vi "Alarm_Pattern_Control.vi"(0 "error in (no error)":errorcluster caption="错误输入（无错误）", 2 "Tilt":bool, 3 "Motion":bool, 4 "State Value":u32) -> (1 "error out":errorcluster caption="错误输出", 5 "Warning Code":u32, 6 "DO0 Pattern":bool)   [LabVIEW 2020]
doc: "PLACEHOLDER: error interface only. Alarm simulation NOT implemented."
panel:
  in  "Red Code":dbl=4.0
  in  "Blue Yellow Code":dbl=3.0
  in  "Yellow Code":dbl=2.0
  in  "Blue Code":dbl=1.0
  in  "No Warning":dbl
  in  "Fast On ms":u32=150
  in  "Fast Period ms":u32=300
  in  "Slow On ms":u32=500
  in  "Slow Period ms":u32=1000
  in  "Beep On ms":u32=200
  in  "Beep Period ms":u32=700
  in  "Blue Beep ms":u32=200
  in  "Code ALARM":u32=3
  in  "Code COUNTDOWN":u32=2
  in  "Code SUSPECT":u32=1
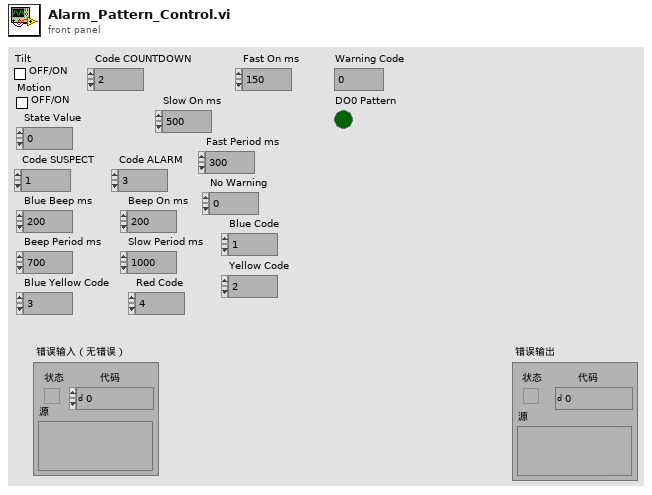
[diagram p1: front panel]
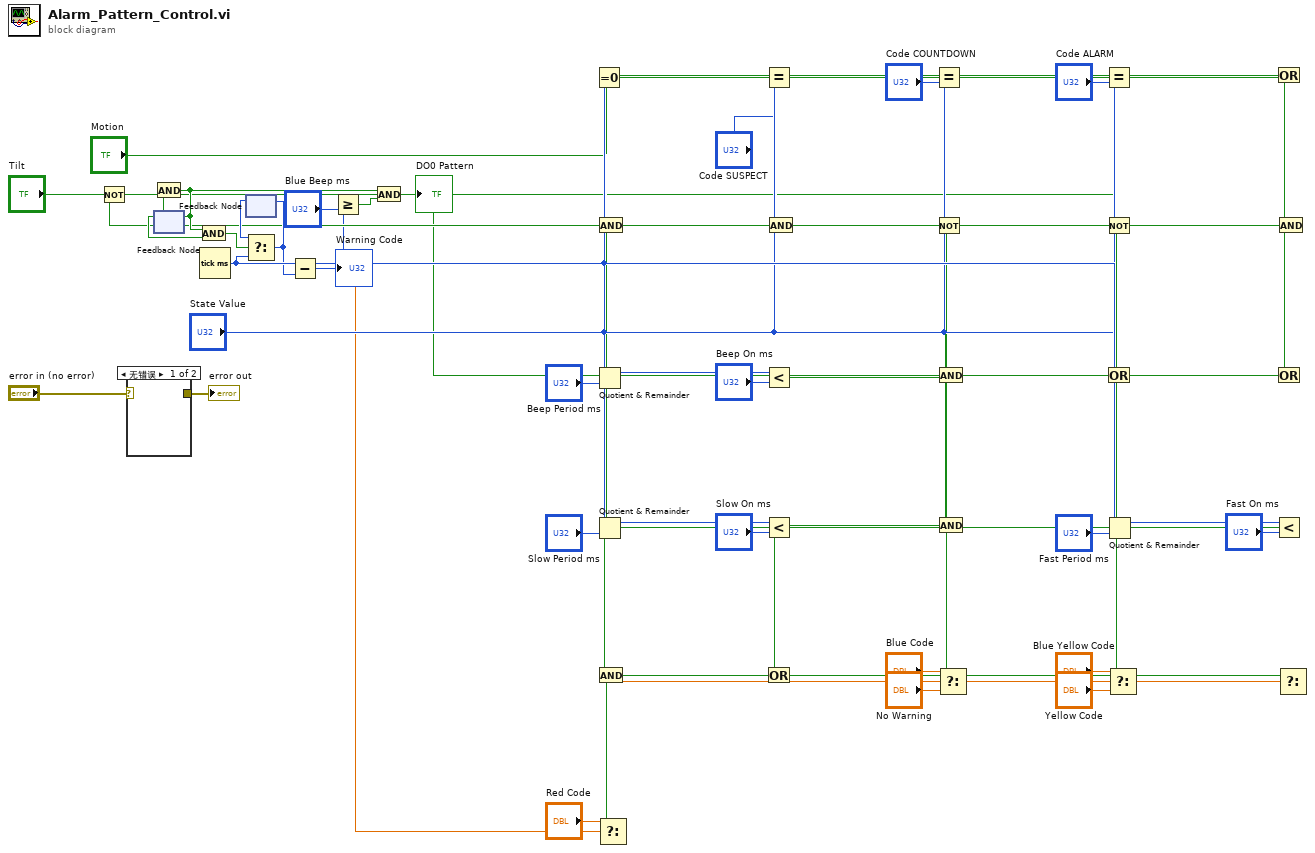
[diagram p0: block diagram]
diagram:
  n1 = case shown="无错误" "error in (no error)" {
    selector: "error in (no error)" -> [_ w57]
    tunnel: [_ w57] -> w55
    frame No Error {
    }
    frame Error {
    }
  }
  "error out" <- w55
  n2 = feedback #1() -> (w52:bool)  [unwired: 1 in]
  n3 = Tick Count (ms)() -> (millisecond timer value=w50:u32)
  n4 = feedback #2() -> (w49:u32)  [unwired: 1 in]
  n5 = Equal To 0?(x="State Value") -> (x = 0?=w40:bool)
  n6 = Quotient & Remainder(x=w50, y="Beep Period ms") -> (x-y*floor(x/y)=w34:u32)  [unwired: 1 out]
  n7 = Quotient & Remainder(x=w50, y="Slow Period ms") -> (x-y*floor(x/y)=w31:u32)  [unwired: 1 out]
  n8 = And(x="Motion", y="Tilt") -> (x .and. y?=w41:bool)
  n9 = Equal?(x="State Value", y="Code SUSPECT") -> (x = y?=w45:bool)
  n10 = Less?(x=w34, y="Beep On ms") -> (x < y?=w33:bool)
  n11 = Less?(x=w31, y="Slow On ms") -> (x < y?=w30:bool)
  n12 = And(x=w40, y=w41) -> (x .and. y?=w39:bool)
  n13 = Equal?(x="State Value", y="Code COUNTDOWN") -> (x = y?=w44:bool)
  n14 = Not(x=w39) -> (.not. x?=w38:bool)
  n15 = Not(x=w38) -> (.not. x?=w54:bool)
  n16 = And(x=w39, y=w54) -> (x .and. y?=w53:bool)
  n17 = feedback-in #1(w53) -> ()
  n18 = And(x=w53, y=w52) -> (x .and. y?=w51:bool)
  n19 = Select(t=w49, s=w51, f=w50) -> (s? t:f=w48:u32)
  n20 = feedback-in #2(w48) -> ()
  n21 = Subtract(x=w50, y=w48) -> (x-y=w37:u32)
  n22 = Greater Or Equal?(x=w37, y="Blue Beep ms") -> (x >= y?=w47:bool)
  n23 = And(x=w53, y=w47) -> (x .and. y?=w36:bool)
  n24 = And(x=w39, y=w30) -> (x .and. y?=w22:bool)
  n25 = Select(t="Blue Code", s=w39, f="No Warning") -> (s? t:f=w20:dbl)
  n26 = Equal?(x="State Value", y="Code ALARM") -> (x = y?=w24:bool)
  n27 = Not(x=w36) -> (.not. x?=w35:bool)
  n28 = Quotient & Remainder(x=w50, y="Fast Period ms") -> (x-y*floor(x/y)=w29:u32)  [unwired: 1 out]
  n29 = Select(t="Blue Yellow Code", s=w39, f="Yellow Code") -> (s? t:f=w18:dbl)
  n30 = Or(x=w44, y=w45) -> (x .or. y?=w32:bool)
  n31 = And(x=w32, y=w33) -> (x .and. y?=w27:bool)
  n32 = Less?(x=w29, y="Fast On ms") -> (x < y?=w28:bool)
  n33 = And(x=w32, y=w28) -> (x .and. y?=w21:bool)
  n34 = Or(x=w21, y=w22) -> (x .or. y?=w19:bool)
  n35 = And(x=w39, y=w35) -> (x .and. y?=w26:bool)
  n36 = Or(x=w26, y=w27) -> (x .or. y?=w25:bool)
  n37 = Or(x=w24, y=w25) -> (x .or. y?=→"DO0 Pattern":bool)
  n38 = Select(t=w18, s=w19, f=w20) -> (s? t:f=w17:dbl)
  n39 = Select(t="Red Code", s=w24, f=w17) -> (s? t:f=→"Warning Code":dbl)
